vi "KYFG Buffer Alloc.vi"(8 "error in (no error)":errorcluster, 10 "frames":u32, 11 "camHandle":u32) -> (0 "error out":errorcluster, 2 "buffHandle":u32, 3 "camHandle out":u32)   [LabVIEW 2023, in "KYFGLib_lv.lvlib"]
doc: "KYFG_API FGSTATUS KYFG_BufferAlloc(CAMHANDLE camHandle, BUFFHANDLE *buffHandle , unsigned int frames);"
uses:
  KYFGLib_lv.lvlib
  KYFGLib.dll
panel:
  in  "buffHandle in":u32
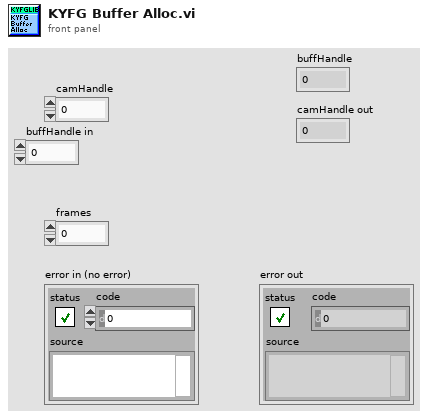
[diagram p1: front panel]
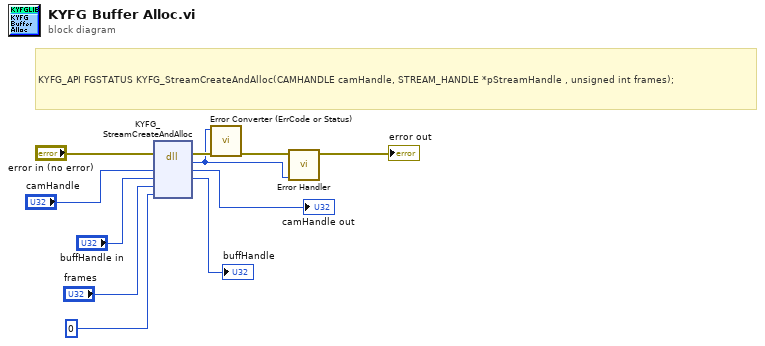
[diagram p0: block diagram]
diagram:
  # "KYFG_API FGSTATUS\tKYFG_StreamCreateAndAlloc(CAMHANDLE camHandle, STREAM_HANDLE *pStreamHandle , unsigned int frames);"
  n1 = dll-call lib="KYFGLib.dll" fn="KYFG_StreamCreateAndAlloc"(error in="error in (no error)", "camHandle"="camHandle", "pStreamHandle"="buffHandle in", "frames"="frames", "streamIndex"=0) -> (error out=w8:errorcluster, "return type"=w4:u32, "camHandle"=→"camHandle out":u32, "pStreamHandle"=→"buffHandle":u32)  [unwired: 4 in, 1 out]
  n2 = call "Error Converter (ErrCode or Status).vi"("error in (no error)"=w8, "error code"=w4) -> ("error out"=w6:errorcluster)  [unwired: 9 in]
  n3 = call "Error Handler.vi"("Return Code"=w4, "Error In"=w6) -> ("Error Out"=→"error out":errorcluster)  [unwired: 9 in]
